vi "Tree.vi"   [LabVIEW 2019, in "LV-Data.PGSQL.lvclass"]
uses:
  LV-Data.PGSQL.lvclass
  API/Write Variable (multirow).vi
  API/Read Variable (integer).vi
  API/Read Variable (double).vi
  API/Write Variable (one-row).vi
  Private/INSERT Multivalue.vi
  API/Read Variable (string).vi
  API/Read Variable (boolean).vi
  Typedefs/Errors--enum.ctl
  Typedefs/Datatypes--enum.ctl
  Typedefs/Configuration--cluster.ctl
  Typedefs/Datatypes--combo.ctl
types:
  T1 = typedef "LV-Data.PGSQL.lvclass/Datatypes--combo.ctl" = string
  T2 = typedef "LV-Data.PGSQL.lvclass/Configuration--cluster.ctl" = cluster{"connection string":string}
  T3 = typedef "LV-Data.PGSQL.lvclass/Datatypes--enum.ctl" = enum16{"double", "string", "json", "integer", "boolean"}
  T4 = typedef "LV-Data.PGSQL.lvclass/Errors--enum.ctl" = enum16{"0: None", "5005: Path Type Not Supported", "5006: Number of Variables", "5007: Number of data points", "5008: Cannot write two data points", "5030: Start and End Times Identical", "5031: Input is not wholly", "5032: Undefined Timestamps", "5033: Bad path or paths", "5040: Invalid Instrument Name", "5050: Column can only hold string", "5051: Column can only hold bool", "5052: Column can only hold double", "5053: Column can only hold int"}
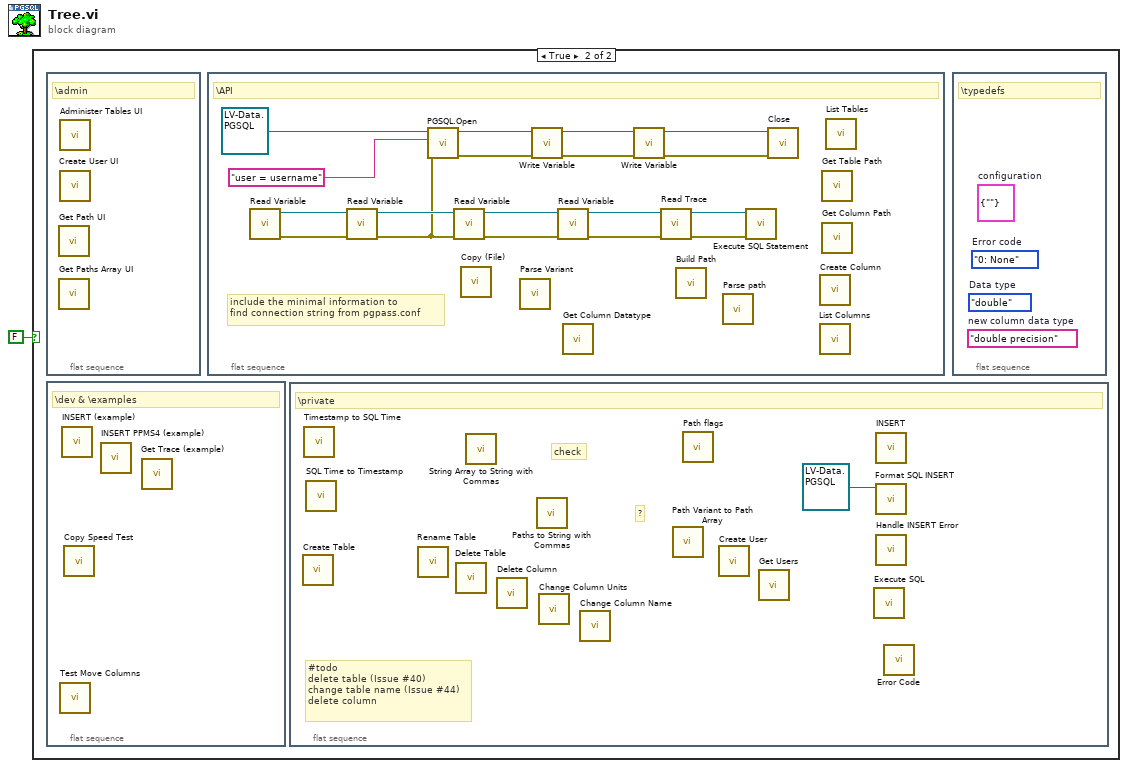
[diagram p0: block diagram]
diagram:
  n1 = case shown="True" FALSE {
    frame False {
    }
    frame True {
      n2 = flat-sequence {
        frame #0 {
          # "\\admin"
          n3 = call "Get Path UI.vi"() -> ()  [unwired: 12 in]
          n4 = call "Get Paths Array UI.vi"() -> ()  [unwired: 10 in, 2 out]
          n5 = call "Administer Tables UI.vi"() -> ()  [unwired: 12 in]
          n6 = call "Create User UI.vi"() -> ()  [unwired: 12 in]
        }
      }
      n7 = flat-sequence {
        frame #0 {
          # "\\dev & \\examples"
          n8 = call "Test Move Columns.vi"() -> ()  [unwired: 11 in, 1 out]
          n9 = call "INSERT (example).vi"() -> ()  [unwired: 12 in]
          n10 = call "Copy Speed Test.vi"() -> ()  [unwired: 12 in]
          n11 = call "INSERT PPMS4 (example).vi"() -> ()  [unwired: 12 in]
          n12 = call "Get Trace (example).vi"() -> ()  [unwired: 12 in]
        }
      }
      n13 = flat-sequence {
        frame #0 {
          # "include the minimal information to\nfind connection string from pgpass.conf"
          # "\\API"
          n14 = call-poly "Read Variable.vi"() -> ("error out"=w13:errorcluster, "Data.PGSQL out"=w12:refnum<class "LV-Data.PGSQL.lvclass">)  [unwired: 6 in, 4 out]
          n15 = call-poly "Read Variable.vi"("error in (no error)"=w13, "Data.PGQL in"=w12) -> ("error out"=w8:errorcluster, "Data.PGSQL out"=w18:refnum<class "LV-Data.PGSQL.lvclass">)  [unwired: 6 in, 2 out]
          n16 = call "PGSQL.Open.vi"("error in (no error)"=w8, "Connection String"="user = username", "Data.PG in"=refnum<class "LV-Data.PGSQL.lvclass"> refnum) -> ("error out"=w9:errorcluster, "Data.PG out"=w10:refnum<class "LV-Data.PGSQL.lvclass">)  [unwired: 7 in]
          n17 = call-poly "Read Variable.vi"("error in (no error)"=w8, "Data.PGQL in"=w18) -> ("error out"=w16:errorcluster, "Data.PGSQL out"=w17:refnum<class "LV-Data.PGSQL.lvclass">)  [unwired: 4 in, 4 out]
          n18 = call "Copy (File).vi"() -> ()  [unwired: 10 in, 2 out]
          n19 = call "Parse Variant.vi"() -> ()  [unwired: 7 in, 5 out]
          n20 = call-poly "Write Variable.vi"("error in (no error)"=w9, "Data.PG in"=w10) -> ("error out"=w6:errorcluster, "Data.PG out"=w5:refnum<class "LV-Data.PGSQL.lvclass">)  [unwired: 6 in, 2 out]
          n21 = call-poly "Read Variable.vi"("error in (no error)"=w16, "Data.PGQL in"=w17) -> ("error out"=w14:errorcluster, "Data.PGSQL out"=w15:refnum<class "LV-Data.PGSQL.lvclass">)  [unwired: 4 in, 4 out]
          n22 = call "Get Column Datatype.vi"() -> ()  [unwired: 9 in, 3 out]
          n23 = call-poly "Write Variable.vi"("error in (no error)"=w6, "Data.PG in"=w5) -> ("error out"=w3:errorcluster, "Data.PG out"=w4:refnum<class "LV-Data.PGSQL.lvclass">)  [unwired: 6 in, 2 out]
          n24 = call "Read Trace.vi"("error in (no error)"=w14, "Data.PGQL in"=w15) -> ("error out"=w19:errorcluster, "Data.PGSQL out"=w20:refnum<class "LV-Data.PGSQL.lvclass">)  [unwired: 5 in, 3 out]
          n25 = call "Build Path.vi"() -> ()  [unwired: 15 in, 1 out]
          n26 = call "Parse path.vi"() -> ()  [unwired: 11 in, 5 out]
          n27 = call "Execute SQL Statement.vi"("error in (no error)"=w19, "Data.PGQL in"=w20) -> ()  [unwired: 7 in, 3 out]
          n28 = call-dynamic "Close.vi"("error in (no error)"=w3, "Data.PG in"=w4) -> ()  [unwired: 8 in, 2 out]
          n29 = call "Create Column.vi"() -> ()  [unwired: 10 in, 2 out]
          n30 = call "List Columns.vi"() -> ()  [unwired: 7 in, 5 out]
          n31 = call "Get Table Path.vi"() -> ()  [unwired: 8 in, 4 out]
          n32 = call "Get Column Path.vi"() -> ()  [unwired: 8 in, 4 out]
          n33 = call "List Tables.vi"() -> ()  [unwired: 8 in, 4 out]
        }
      }
      n34 = flat-sequence {
        frame #0 {
          # "#todo\ndelete table (Issue #40)\nchange table name (Issue #44)\ndelete column"
          # "check"
          # "?"
          # "\\private"
          n35 = call "Create Table.vi"() -> ()  [unwired: 10 in, 2 out]
          n36 = call "Timestamp to SQL Time.vi"() -> ()  [unwired: 11 in, 1 out]
          n37 = call "SQL Time to Timestamp.vi"() -> ()  [unwired: 1 in, 1 out]
          n38 = call "Rename Table.vi"() -> ()  [unwired: 9 in, 3 out]
          n39 = call "Delete Table.vi"() -> ()  [unwired: 10 in, 2 out]
          n40 = call "String Array to String with Commas.vi"() -> ()  [unwired: 1 in, 1 out]
          n41 = call "Delete Column.vi"() -> ()  [unwired: 10 in, 2 out]
          n42 = call "Paths to String with Commas.vi"() -> ()  [unwired: 10 in, 2 out]
          n43 = call "Change Column Units.vi"() -> ()  [unwired: 10 in, 2 out]
          n44 = call "Change Column Name.vi"() -> ()  [unwired: 10 in, 2 out]
          n45 = call "Path Variant to Path Array.vi"() -> ()  [unwired: 10 in, 2 out]
          n46 = call "Path flags.vi"() -> ()  [unwired: 11 in, 5 out]
          n47 = call "Create User.vi"() -> ()  [unwired: 10 in, 2 out]
          n48 = call "Get Users.vi"() -> ()  [unwired: 9 in, 3 out]
          n49 = call "Execute SQL.vi"() -> ()  [unwired: 8 in, 4 out]
          n50 = call "INSERT.vi"() -> ()  [unwired: 8 in, 4 out]
          n51 = call "Format SQL INSERT.vi"("LV-Data.PGSQL in"=refnum<class "LV-Data.PGSQL.lvclass"> refnum ("Data.PG in")) -> ()  [unwired: 7 in, 4 out]
          n52 = call "Handle INSERT Error.vi"() -> ()  [unwired: 9 in, 3 out]
          n53 = call "Error Code.vi"() -> ()  [unwired: 11 in, 1 out]
        }
      }
      n54 = flat-sequence {
        frame #0 {
          (unwired) T1 "double precision"  # new column data type
          (unwired) T2 {"connection string"=""}  # configuration
          (unwired) Datatypes--enum."double"  # Data type
          (unwired) Errors--enum."0: None"  # Error code
          # "\\typedefs"
        }
      }
    }
  }
